vi "Start Log.vi"(7 "Node Name":string, 8 "error in (no error)":errorcluster, 9 "Time Stamp":timestamp, 10 "Folder":path, 11 "Event Reporter Module in":refnum<class "Event Reporter Module.lvclass">) -> (0 "error out":errorcluster, 3 "Event Reporter Module out":refnum<class "Event Reporter Module.lvclass">)   [LabVIEW 2020, in "Volatus.lvlib" / "Event Reporter Module.lvclass"]
uses:
  Event Reporter Module.lvclass
  lv-cdm/CDM-Config/ISO8601 Config.ctl
  lv-cdm/CDM-Config/Format.ctl
  lv-cdm/CDM-Config/Precision.ctl
  lv-cdm/CDM-Config/Timezone.ctl
  Event Reporter Module.lvclass/Event Reporter Module.ctl
  lv-cdm/CDM-Config/ISO-8601 Format Strings.vi
  lv-cdm/CDM-Config/CDM-Config.lvlib
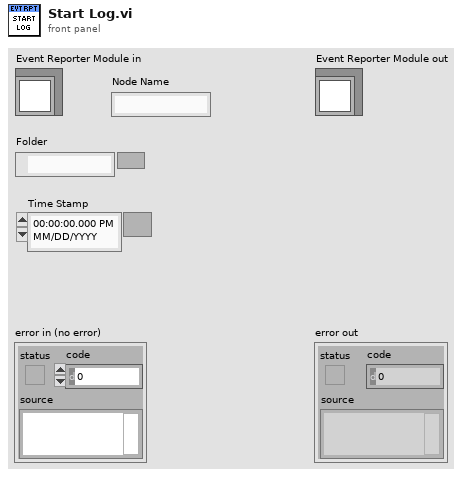
[diagram p1: front panel]
types:
  T1 = enum16{"open", "replace", "create", "open or create", "replace or create", "replace or create with confirmation"}
  T2 = typedef "CDM-Config.lvlib/ISO8601 Config.ctl" = cluster{"Format":T3, "Precision":T4, "Timezone":T5}
  T3 = typedef "CDM-Config.lvlib/Format.ctl" = enum16{"Extended", "Basic"}
  T4 = typedef "CDM-Config.lvlib/Precision.ctl" = enum16{"Millisecond", "Second", "Minute", "Hour", "Day"}
  T5 = typedef "CDM-Config.lvlib/Timezone.ctl" = enum16{"UTC", "Local"}
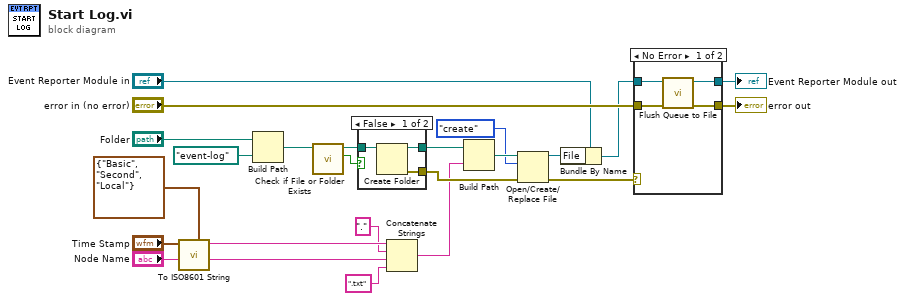
[diagram p0: block diagram]
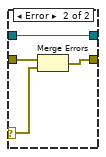
[diagram p2: hidden frame]
diagram:
  n1 = call "To ISO8601 String.vi"("Format Config"=T2 {"Format"=enum."Basic", "Precision"=enum."Second", "Timezone"=enum."Local"}, "Time Stamp"="Time Stamp") -> ("ISO 8601"=w3:string)  [unwired: 9 in]
  n2 = Build Path(base path="Folder", name or relative path=path "event-log") -> (appended path=w17:path)
  n3 = call <vilib>:"Check if File or Folder Exists.vi"("path"=w17) -> ("file or folder exists?"=w16:bool, "dup path"=w15:path)  [unwired: 8 in, 1 out]
  n4 = case shown="False" w16 {
    tunnel: w15 -> [w26 w27]
    tunnel: [w25 w27] -> w10
    tunnel: [w24 _] -> w22
    frame False {
      n5 = Create Folder(path (use dialog)=w26) -> (created path=w25:path, error out=w24:errorcluster)  [unwired: 2 in, 1 out]
    }
    frame True {
    }
  }
  n6 = Concatenate Strings(w3, "." ("string"), "Node Name", ".txt" ("string")) -> (w11:string)
  n7 = Build Path(base path=w10, name or relative path=w11) -> (appended path=w14:path)
  n8 = Open/Create/Replace File(file path (use dialog)=w14, error in=w22, operation (0:open)=T1."create") -> (refnum out=w9:refnum<file>, error out=w8:errorcluster)  [unwired: 3 in, 1 out]
  n9 = Bundle By Name(cluster="Event Reporter Module in", "File"=w9) -> (w6:refnum<class "Event Reporter Module.lvclass">)
  n10 = case shown="No Error" w8 {
    selector: w8 -> [_ w33]
    tunnel: [w29 w35] -> w7
    tunnel: w6 -> [w31 w35]
    tunnel: "error in (no error)" -> [w30 w34]
    tunnel: [w28 w32] -> w5
    frame No Error {
      n11 = call "Flush Queue to File.vi"("error in (no error)"=w30, "Event Reporter Module in"=w31) -> ("error out"=w28:errorcluster, "Event Reporter Module out"=w29:refnum<class "Event Reporter Module.lvclass">)  [unwired: 8 in]
    }
    frame Error {
      n12 = Merge Errors(w34, w33) -> (w32:errorcluster)
    }
  }
  "error out" <- w5
  "Event Reporter Module out" <- w7
